vi "power_measurement.vi"(7 "Measured Power Chart Ref":refnum<vi>, 8 "error in":errorcluster, 9 "Measured Power Ref":refnum<vi>, 10 "Stop Ref":refnum<vi>, 11 "OphirLMMeasurementLib.ICoLMMeasurement2":refnum<k7>) -> (0 "error out":errorcluster)   [LabVIEW 2025, in "tSNIP.lvlib"]
uses:
  tSNIP.lvlib
panel:
  out "Measured Power":cluster{"Value":dbl, "Units":dbl}={"Value"=0.0, "Units"=0.001} {"Units" items=["mW"=0.001, "W"=1.0]; "Value" min=0.0 step=50.0}
  out "Device S/Ns":string[](array[string])
  out "Readings":T1(array[cluster]) {"value" format="%#_6p"; "timestamp" format="%#.3f"}
  out "Selected device S/N":string
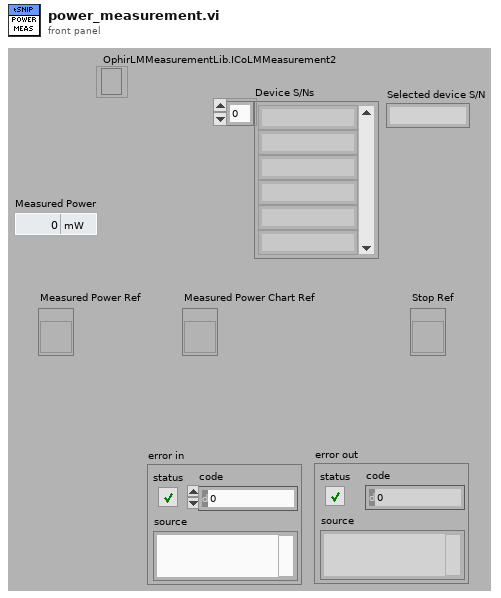
[diagram p1: front panel]
types:
  T1 = cluster{"value":dbl, "timestamp":dbl, "status":i32}[]
  T2 = cluster{"value":dbl, "timestamp":dbl, "status":i32}
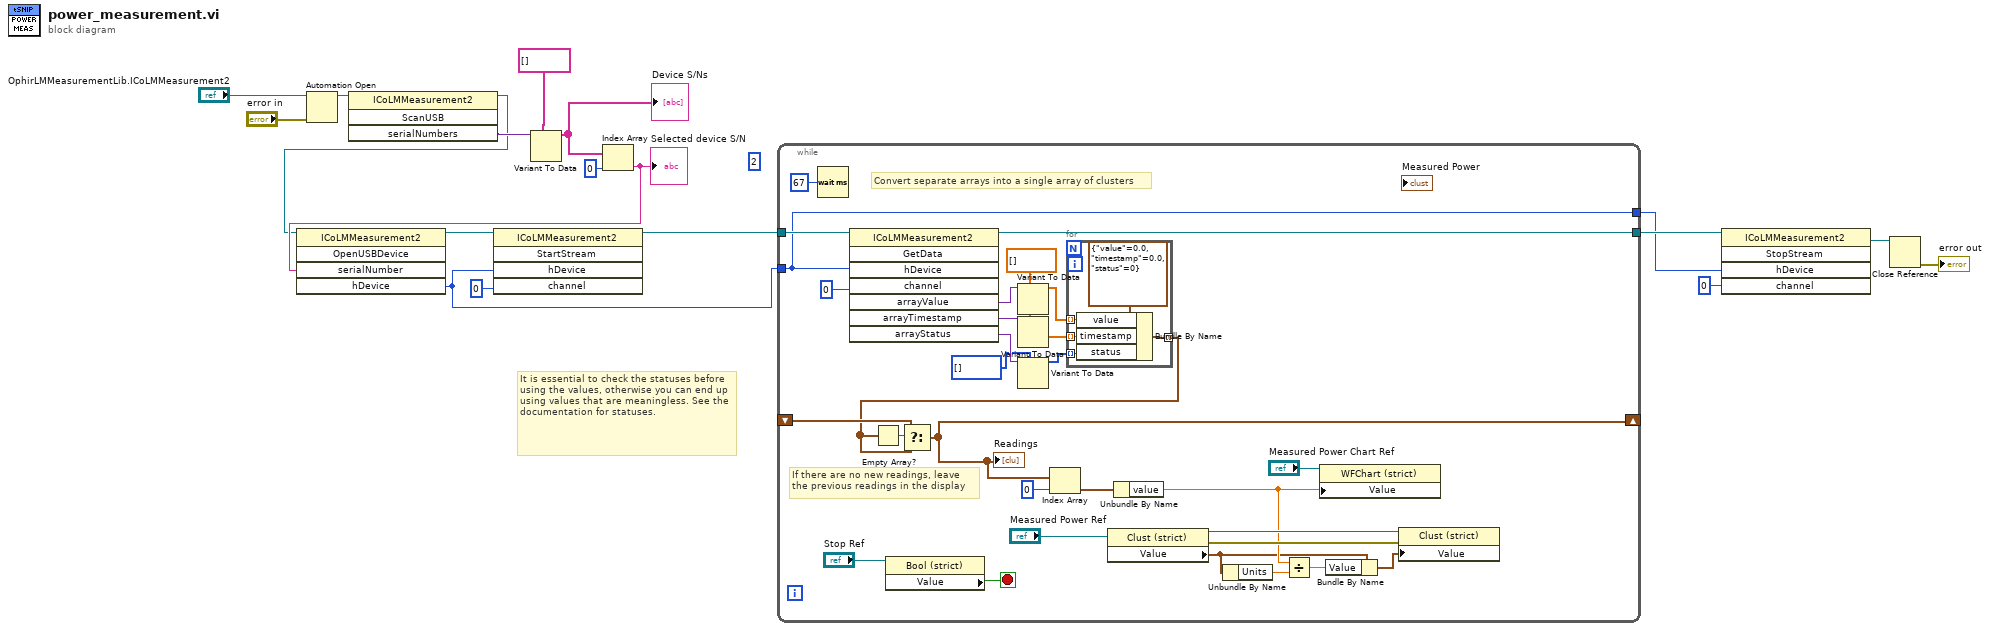
[diagram p0: block diagram]
diagram:
  (unwired) 2
  # "It is essential to check the statuses before using the values, otherwise you can end up using values that are meaningless. See the documentation for statuses."
  n1 = Automation Open(error in (no error)="error in", Automation Refnum="OphirLMMeasurementLib.ICoLMMeasurement2") -> (Automation Refnum=w17:refnum<k7>)  [unwired: 2 in, 1 out]
  n2 = invoke class="ICoLMMeasurement2" method="ScanUSB"(reference=w17) -> (reference out=w11:refnum<k7>, "serialNumbers"=w16:variant)  [unwired: 3 in, 2 out]
  n3 = Variant To Data(type=string[] [], Variant=w16) -> (data=w15:string[])  [unwired: 1 in, 1 out]
  "Device S/Ns" <- w15
  n4 = Index Array(array=w15, index=0) -> (element=w12:string)
  "Selected device S/N" <- w12
  n5 = invoke class="ICoLMMeasurement2" method="OpenUSBDevice"(reference=w11, "serialNumber"=w12) -> (reference out=w10:refnum<k7>, "hDevice"=w8:i32)  [unwired: 3 in, 3 out]
  n6 = invoke class="ICoLMMeasurement2" method="StartStream"(reference=w10, "hDevice"=w8, "channel"=0) -> (reference out=w9:refnum<k7>)  [unwired: 2 in, 4 out]
  n7 = while {
    tunnel: w9 -> [w47]
    tunnel: w8 -> [w44]
    tunnel: [w45] -> w6
    tunnel: [w44] -> w5
    shift-right: [w32] -> _
    shift-left: _ -> [w35]
    stop <- w28 stop-if-true
    w43 = dbl[] []
    # "Convert separate arrays into a single array of clusters"
    # "If there are no new readings, leave\nthe previous readings in the display"
    n8 = Wait (ms)(milliseconds to wait=u32 67) -> ()  [unwired: 1 out]
    n9 = invoke class="ICoLMMeasurement2" method="GetData"(reference=w47, "hDevice"=w44, "channel"=0) -> (reference out=w45:refnum<k7>, "arrayValue"=w42:variant, "arrayTimestamp"=w41:variant, "arrayStatus"=w40:variant)  [unwired: 5 in, 4 out]
    n10 = property class="Bool (strict)"(reference="Stop Ref") -> ("Value"=w28:bool)  [unwired: 1 in, 2 out]
    n11 = Variant To Data(type=w43, Variant=w42) -> (data=w39:dbl[])  [unwired: 1 in, 1 out]
    n12 = Variant To Data(type=w43, Variant=w41) -> (data=w38:dbl[])  [unwired: 1 in, 1 out]
    n13 = Variant To Data(type=i32[] [], Variant=w40) -> (data=w37:i32[])  [unwired: 1 in, 1 out]
    n14 = for {
      tunnel: w39 -> [w52] mode=indexing
      tunnel: w38 -> [w51] mode=indexing
      tunnel: w37 -> [w50] mode=indexing
      tunnel: [w49] -> w33 mode=indexing
      n15 = Bundle By Name(cluster=T2 {"value"=0.0, "timestamp"=0.0, "status"=0}, "value"=w52, "timestamp"=w51, "status"=w50) -> (w49:T2)
    }
    n16 = Empty Array?(array=w33) -> (empty?=w34:bool)
    n17 = Select(t=w35, s=w34, f=w33) -> (s? t:f=w32:T1)
    "Readings" <- w32
    n18 = Index Array(array=w32, index=0) -> (element=w30:T2)
    n19 = property class="Clust (strict)"(reference="Measured Power Ref") -> (reference out=w25:refnum<vi>, error out=w24:errorcluster, "Value"=w20:cluster{"Value":dbl, "Units":dbl})  [unwired: 1 in]
    n20 = Unbundle By Name(w30) -> ("value"=w22:dbl)
    n21 = Unbundle By Name(w20) -> ("Units"=w23:dbl)
    n22 = Divide(x=w22, y=w23) -> (x/y=w21:dbl)
    n23 = property class="WFChart (strict)"(reference="Measured Power Chart Ref", "Value"=w22) -> ()  [unwired: 1 in, 2 out]
    n24 = Bundle By Name(cluster=w20, "Value"=w21) -> (w19:cluster{"Value":dbl, "Units":dbl})
    n25 = property class="Clust (strict)"(reference=w25, error in=w24, "Value"=w19) -> ()  [unwired: 2 out]
  }
  n26 = invoke class="ICoLMMeasurement2" method="StopStream"(reference=w6, "hDevice"=w5, "channel"=0) -> (reference out=w3:refnum<k7>)  [unwired: 2 in, 4 out]
  n27 = Close Reference(reference=w3) -> (error out=→"error out":errorcluster)  [unwired: 1 in]
